vi "Consumer.vi"(8 "error in (no error)":errorcluster, 9 "Data":variant, 10 "Case ID":string, 11 "Scheduler in":refnum<class "Scheduler.lvclass">) -> (0 "error out":errorcluster, 3 "Scheduler out":refnum<class "Scheduler.lvclass">)   [LabVIEW 2020, in "Scheduler.lvlib" / "Scheduler.lvclass"]
uses:
  Scheduler.lvclass
  C:/LabVIEW Code/CIRCUS/TALOS/TALOS_PPL.lvlibp/Father of all uServices/Father of all uServices/Father of all uServices.lvclass
  Scheduler Consumer Case Selector.ctl
  Add RUN Output Data Packet.ctl
  Run Utilities/Schedule Block/Schedule Block.lvclass
  Scheduler.lvclass/Scheduler.ctl
  Run Utilities/Sequence of SBlocks/Sequence of SBlocks.lvclass
  Run Utilities/TypeDefs/Synchronize FPGA Cluster.ctl
  Append Options.ctl
  Run Utilities/TypeDefs/Messages/Schedules With Sync Mask Message.ctl
  Run Utilities/Schedule/Schedule.lvclass
  Run Utilities/TypeDefs/Messages/Append Schedule Message.ctl
  Selection.ctl
  cc9169f9-c1ee-4f38-a286-790ff9248fc5.vi
  7fb8f17a-4757-400c-9638-1f609eaaf37f.vi
  TALOS/TALOS_PPL.lvlibp/Support VIs/Global Memory.vi
  Add RUN Window.vi
  TALOS/TALOS_PPL.lvlibp/Father of all uServices/Father of all uServices/Children Methods/Get GUI Item Value - Variant.vi
  TALOS/TALOS_PPL.lvlibp/Support VIs/Global Constants.vi
  <vilib>/Comparison/Equal/Equal Functor/Equal Functor.lvclass
  TALOS/TALOS_PPL.lvlibp/Father of all uServices/Father of all uServices/Father of all uServices.lvclass
  Run Utilities/Run Utilities.lvlib
  TALOS/TALOS_PPL.lvlibp
  C:/LabVIEW Code/CIRCUS/TALOS/TALOS_PPL.lvlibp/Ancestor/Ancestor/Ancestor.lvclass
  C:/LabVIEW Code/CIRCUS/TALOS/Actor Framework.lvlibp/1abvi3w/vi.lib/ActorFramework/Actor/Actor.lvclass
  C:/LabVIEW Code/CIRCUS/CIRCUS uServices et al/Scheduler/Scheduler.lvclass
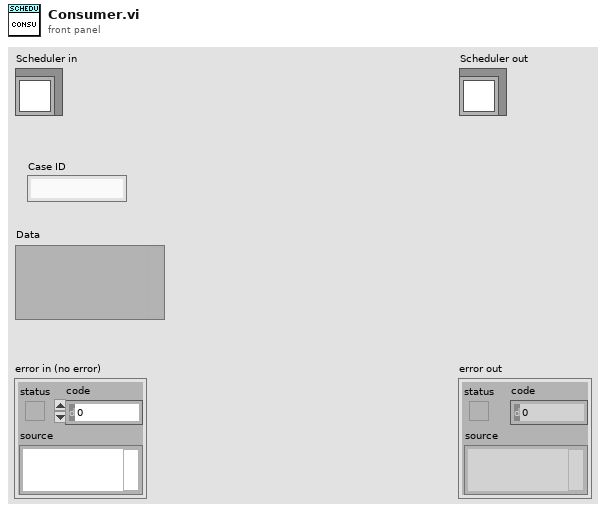
[diagram p1: front panel]
types:
  T1 = typedef "Scheduler.lvlib/Scheduler.lvclass/Scheduler Consumer Case Selector.ctl" = enum16{"Add SBlock", "Update GUI", "Move SBlock", "Select SBlock", "Update Cont.", "Load", "Save", "Reset", "Send to Tamer", "Edit SBlock", "Duplicate SBlock", "Delete SBlock", "Update SBlock", "Init", "Split/Combine Schedules", "Reschedule", "Load Parameters"}
  T2 = enum8{"Enabled", "Disabled", "Disabled and Grayed Out"}
  T3 = typedef "Scheduler.lvlib/Scheduler.lvclass/Add RUN Output Data Packet.ctl" = cluster{"Index":i32, "Schedule Block":refnum<class "Schedule Block.lvclass">}
  T4 = enum32{"Invalid", "Standard", "Closed", "Hidden", "Minimized", "Maximized"}
  T5 = typedef "Scheduler.lvlib/Scheduler.lvclass/Append Options.ctl" = enum16{"New session", "Append to bottom", "Append to top"}
  T6 = typedef "Run Utilities.lvlib/Schedules With Sync Mask Message.ctl" = cluster{"Schedules":refnum<class "Schedule.lvclass">[], "Synchronised":T7[]}
  T7 = typedef "Run Utilities.lvlib/Synchronize FPGA Cluster.ctl" = cluster{"Status":bool, "FPGA Name":string}
  T8 = typedef "Run Utilities.lvlib/Append Schedule Message.ctl" = cluster{"List of FPGAs":set{string}, "Schedules":refnum<class "Schedule.lvclass">[], "To Top?":bool}
  T9 = typedef "Scheduler.lvlib/Scheduler.lvclass/Selection.ctl" = cluster{"Row":i32, "Column":i32}
  T10 = typedef "Run Utilities.lvlib/Sequence of SBlocks.lvclass/Sequence of SBlcoks - GUI.ctl" = cluster{"Total number of scripts":i32, "Time":string, "Sequence of SBlocks":T11[], "Continuous":bool}
  T11 = typedef "Run Utilities.lvlib/Schedule Block.lvclass/Schedule Block - simplified GUI.ctl" = cluster{"Bcg Color":u32, "Index":i32, "No. of runs":i32, "Script name":string, "FPGA name":string, "Parameters":string, "Repetitions":i32}
  T12 = cluster{"SBlock Index":i32, "Sequence Index":i32}
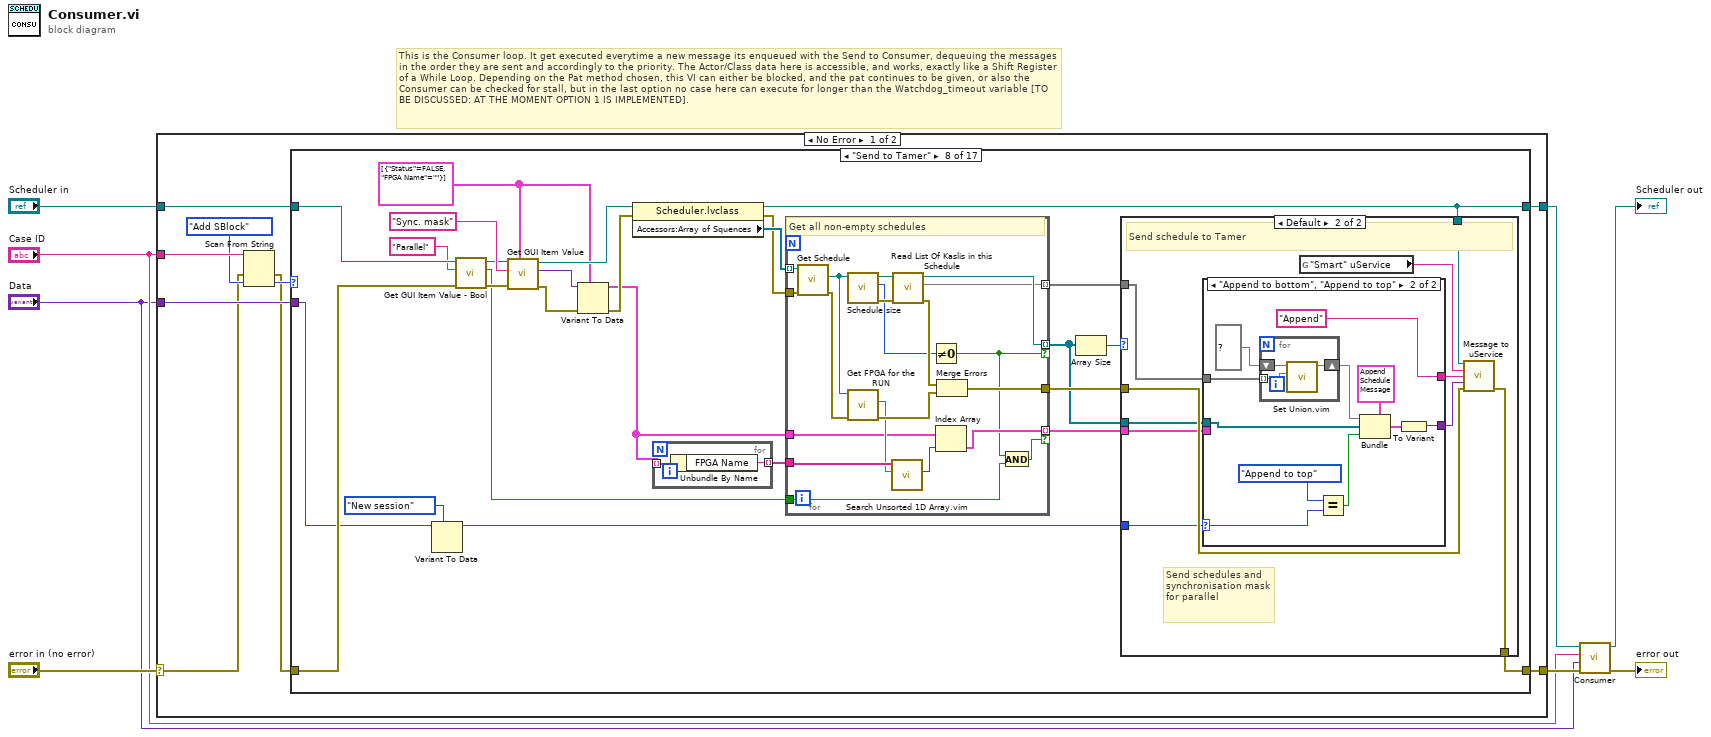
[diagram p0: block diagram]
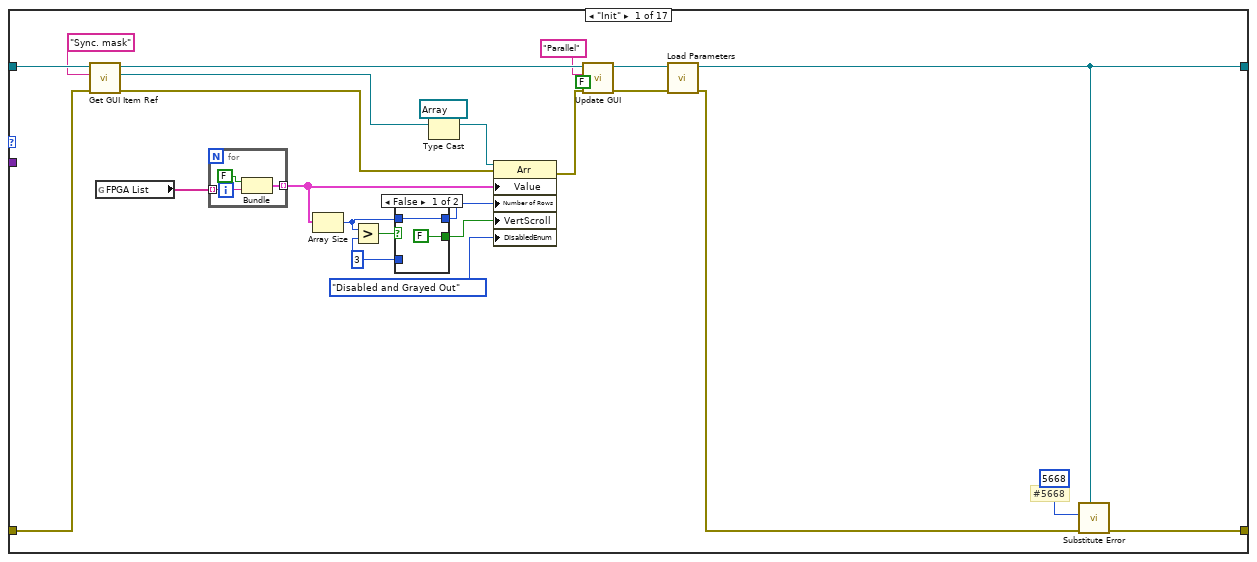
[diagram p2: hidden frame]
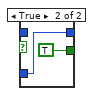
[diagram p3: hidden frame]
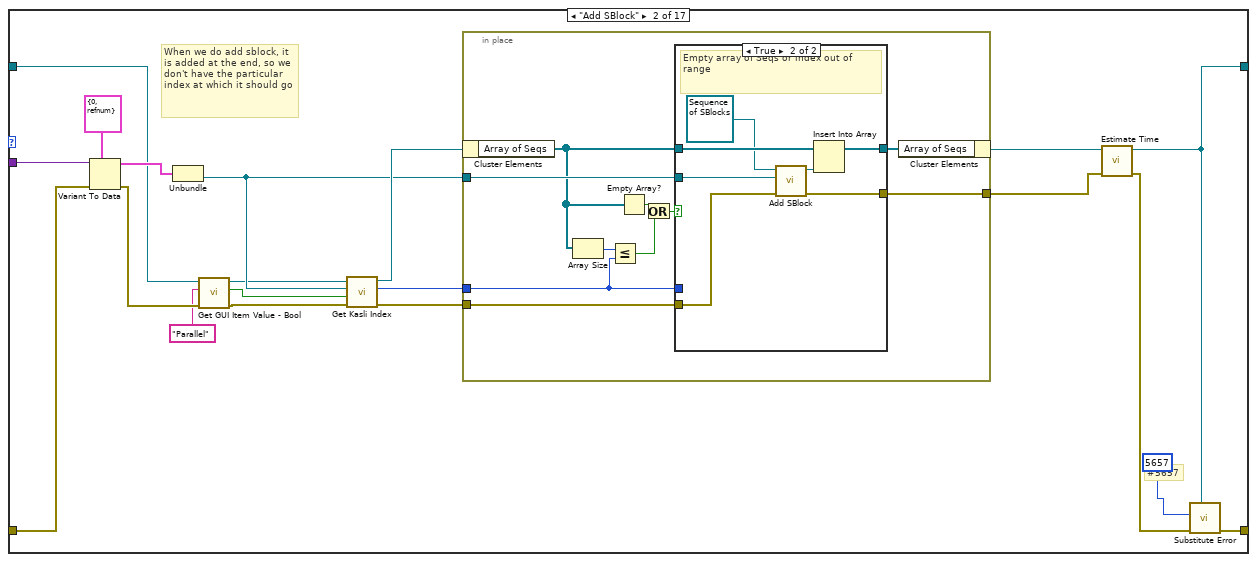
[diagram p4: hidden frame]
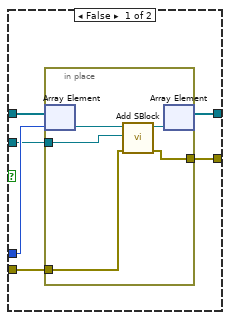
[diagram p5: hidden frame]
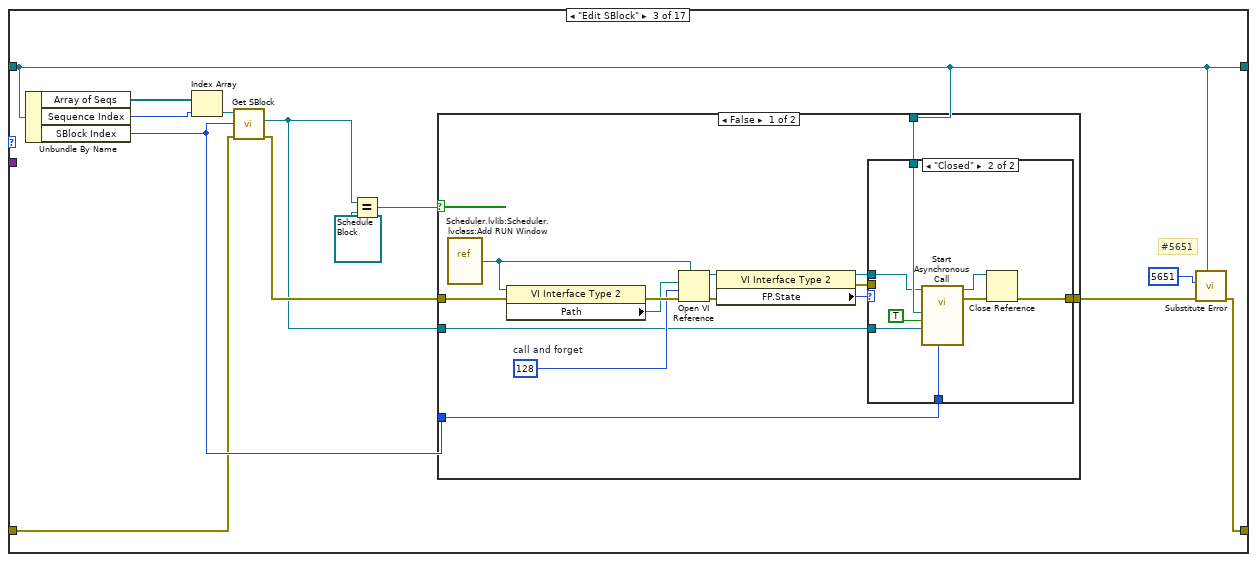
[diagram p6: hidden frame]
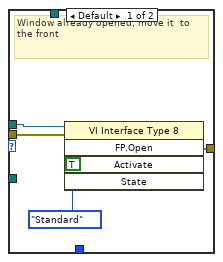
[diagram p7: hidden frame]
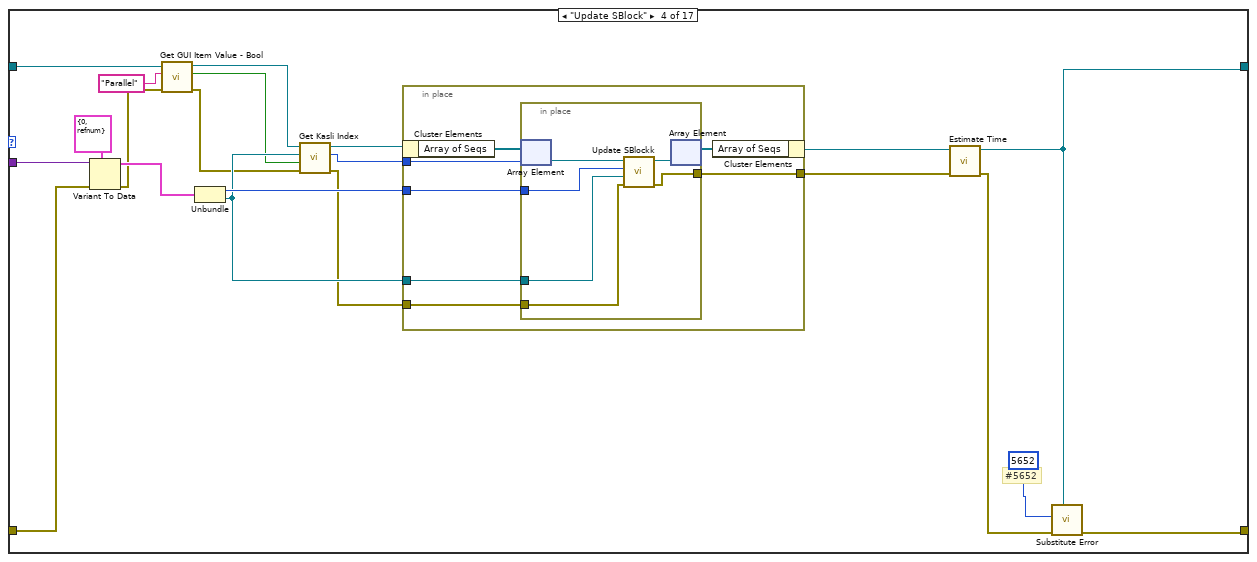
[diagram p9: hidden frame]
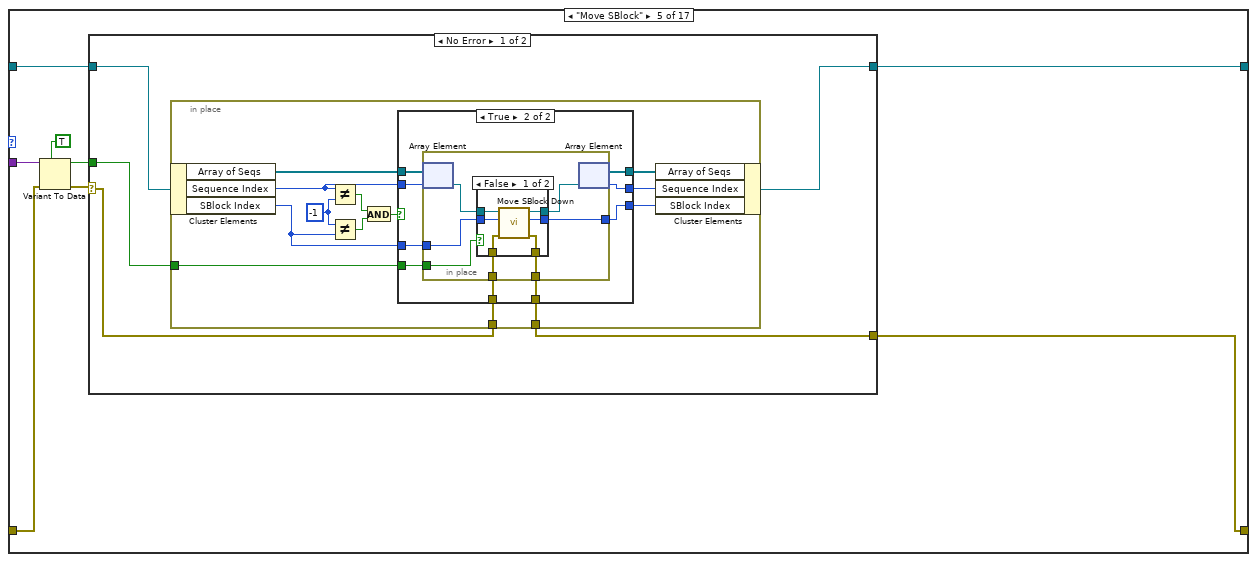
[diagram p10: hidden frame]
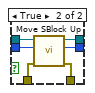
[diagram p12: hidden frame]
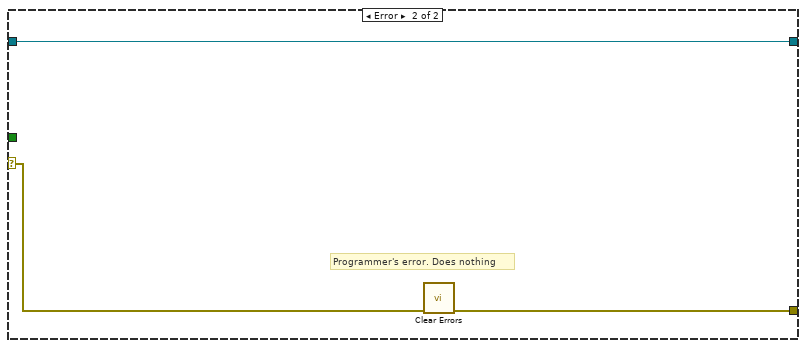
[diagram p13: hidden frame]
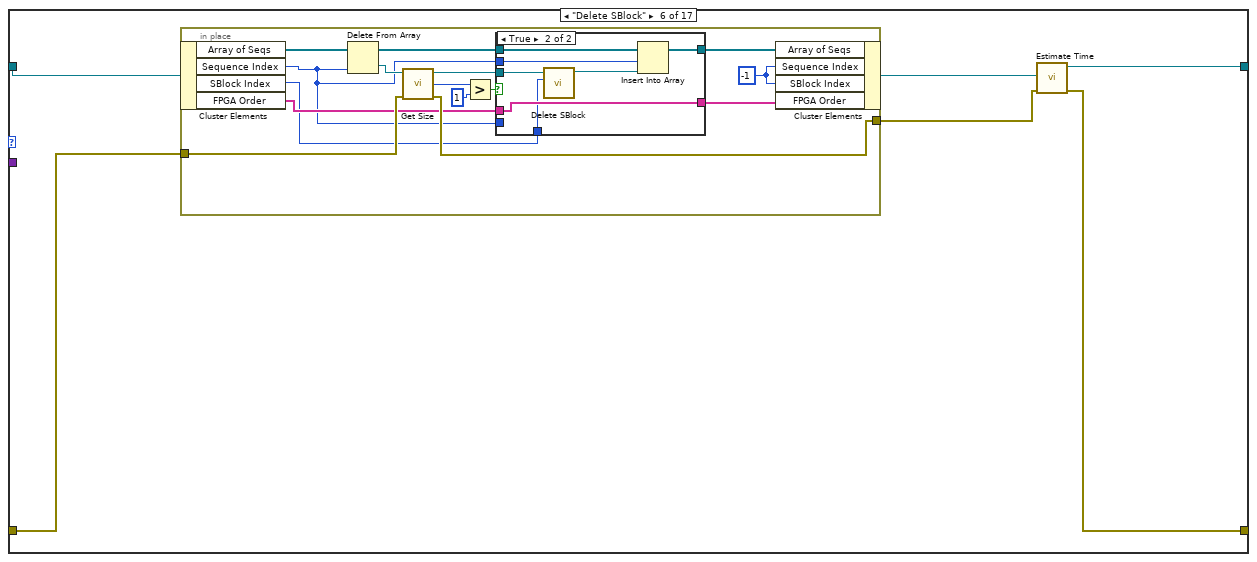
[diagram p14: hidden frame]
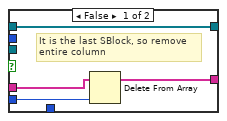
[diagram p15: hidden frame]
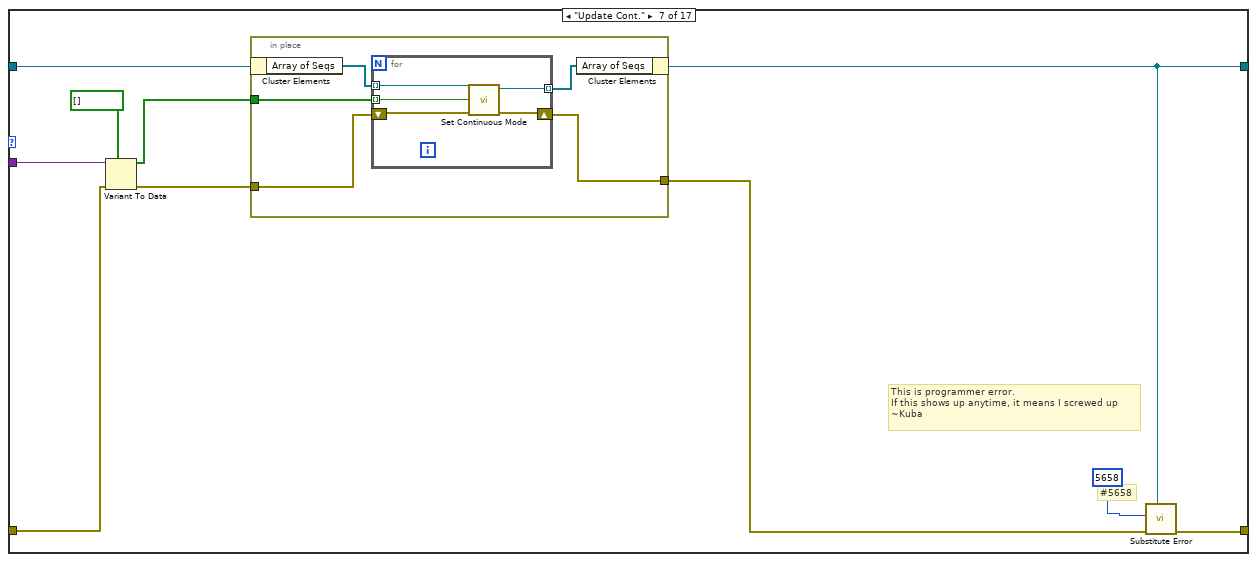
[diagram p16: hidden frame]
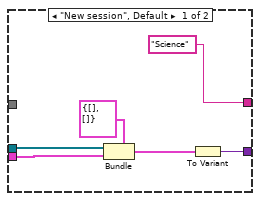
[diagram p18: hidden frame]
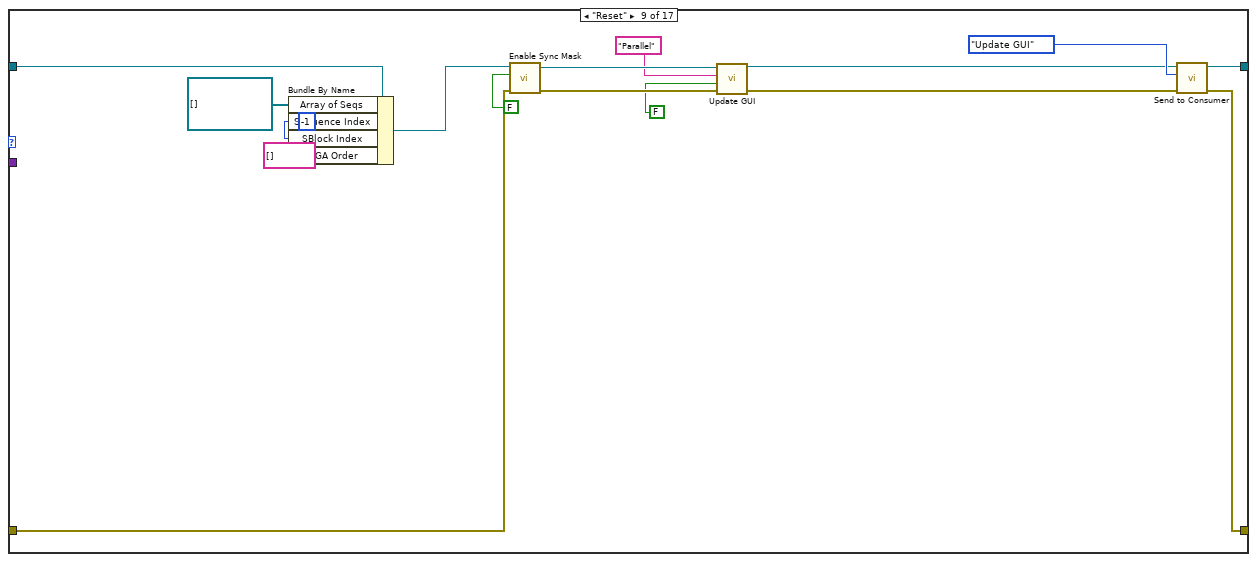
[diagram p19: hidden frame]
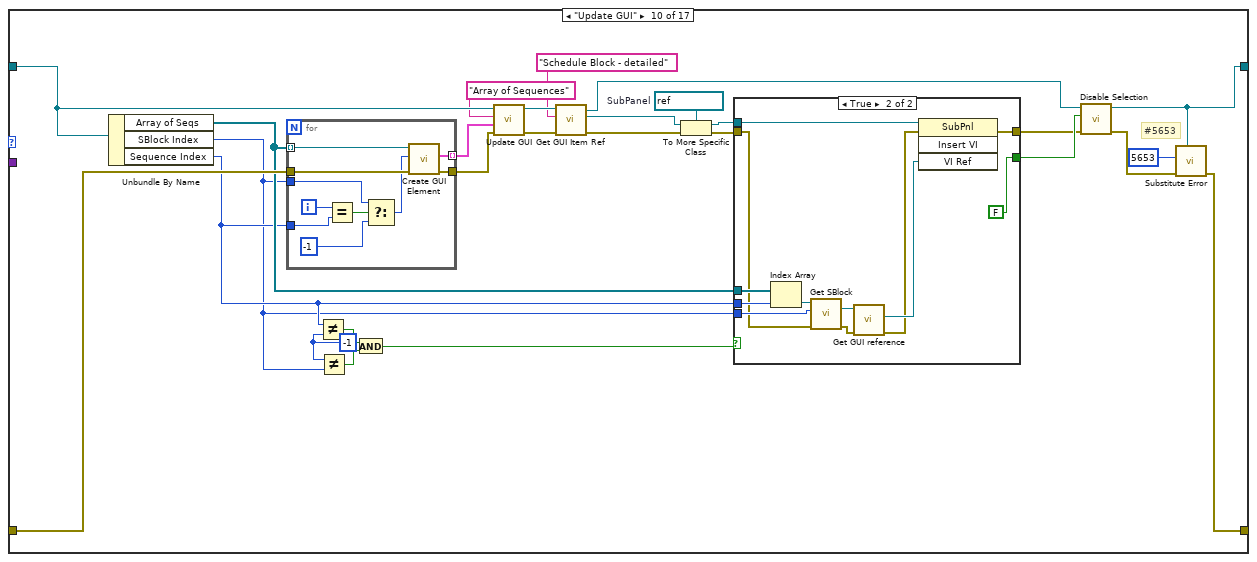
[diagram p20: hidden frame]
diagram:
  # "This is the Consumer loop. It get executed everytime a new message its enqueued with the Send to Consumer, dequeuing the messages in the order they are sent and accordingly to the priority. The Actor/Class data here is accessible, and works, exactly like a Shift Register of a While Loop. Depending on the Pat method chosen, this VI can either be blocked, and the pat continues to be given, or also the Consumer can be checked for stall, but in the last option no case here can execute for longer than the Watchdog_timeout variable [TO BE DISCUSSED: AT THE MOMENT OPTION 1 IS IMPLEMENTED]."
  n1 = case shown="No Error" "error in (no error)" {
    selector: "error in (no error)" -> [w11 w623]
    tunnel: [w10 w624] -> w3
    tunnel: "Scheduler in" -> [w17 w624]
    tunnel: [w15 w623] -> w6
    tunnel: "Case ID" -> [w14 _]
    tunnel: "Data" -> [w16 _]
    frame No Error {
      n2 = Scan From String(input string=w14, error in=w11, default 1=Scheduler_Consumer_Case_Selector."Add SBlock" ("Consumer Case Selector")) -> (error out=w9:errorcluster, output 1=w12:T1)  [unwired: 2 in, 2 out]
      n3 = case shown="\"Send to Tamer\"" w12 {
        tunnel: w17 -> [w35 w55 w108 w143 w180 w239 w275 w305 w371 w405 w437 w489 w517 w540 w586 w616 w621]
        tunnel: w16 -> [_ w69 _ w159 w178 _ w274 w290 _ _ w435 w488 _ w539 w588 w618 _]
        tunnel: [w20 w61 w110 w150 w173 w235 w270 w310 w379 w407 w439 w491 w511 w532 w585 w609 w619] -> w15
        tunnel: w9 -> [w34 w66 w103 w155 w174 w238 w273 w304 w368 w404 w434 w487 w518 w537 w587 w613 w622]
        tunnel: [w19 w58 w108 w147 w179 w236 w269 w309 w380 w394 w438 w490 w512 w536 w583 w610 w620] -> w10
        frame "Init" {
          w37 = 3 ("y")
          # "#5668"
          n4 = call "Get GUI Item Ref.vi"("error in (no error)"=w34, "FP Item Name"="Sync. mask", "uService Template in"=w35) -> ("error out"=w29:errorcluster, "Ctl Refnum"=w33:refnum<vi>, "uService Template out"=w28:refnum<class "Scheduler.lvclass">)  [unwired: 6 in]
          n5 = global read "Global Memory.vi" "FPGA List"() -> (w22:string[])
          n6 = for {
            tunnel: w22 -> [w48] mode=indexing
            tunnel: [w47] -> w36 mode=indexing
            n7 = Bundle(FALSE, "AEgIS PCs List"=w48) -> (w47:cluster{bool, "AEgIS PCs List":string})  [unwired: 1 in]
          }
          n8 = Array Size(array=w36) -> (size(s)=w39:i32)
          n9 = Greater?(x=w39, y=w37) -> (0:w42:bool)
          n10 = case shown="False" w42 {
            tunnel: [w43 w45] -> w41
            tunnel: [FALSE TRUE] -> w40
            tunnel: w39 -> [w43 _]
            tunnel: w37 -> [_ w45]
            frame False {
            }
            frame True {
            }
          }
          n11 = Type Cast(type=refnum<vi> refnum ("reference"), x=w33) -> (*(type *) &x=w31:refnum<vi>)
          n12 = property class="Arr"(reference=w31, error in=w29, "Value"=w36, "Number of Rows"=w41, "VertScroll"=w40, "DisabledEnum"=T2."Disabled and Grayed Out" ("Disabled")) -> (error out=w27:errorcluster)  [unwired: 1 out]
          n13 = call "Update GUI.vi"("error in (no error)"=w27, "Data"=FALSE, "GUI Item Name"="Parallel", "uService Template in"=w28) -> ("error out"=w24:errorcluster, "uService Template out"=w23:refnum<class "Scheduler.lvclass">)  [unwired: 6 in]
          n14 = call-dynamic "Load Parameters.vi"("error in (no error)"=w24, "Scheduler in"=w23) -> ("error out"=w21:errorcluster, "Scheduler out"=w19:refnum<class "Scheduler.lvclass">)  [unwired: 8 in]
          n15 = call "Substitute Error.vi"("LabVIEW Object"=w19, "error in (no error)"=w21, "Error Code"=5668) -> ("error out"=w20:errorcluster)  [unwired: 8 in]
        }
        frame "Add SBlock" {
          # "When we do add sblock, it is added at the end, so we don't have the particular index at which it should go"
          # "#5657"
          n16 = Variant To Data(error in=w66, type=T3 {"Index"=0, "Schedule Block"=refnum} ("Cluster"), Variant=w69) -> (data=w67:T3, error out=w54:errorcluster)
          n17 = Unbundle(w67) -> ("Schedule Block"=w62:refnum<class "Schedule Block.lvclass">)  [unwired: 1 out]
          n18 = call "Get GUI Item Value - Bool.vi"("error in (no error)"=w54, "FP Item Name"="Parallel", "uService Template in"=w55) -> ("error out"=w53:errorcluster, "Value"=w51:bool, "uService Template out"=w52:refnum<class "Scheduler.lvclass">)  [unwired: 6 in]
          n19 = call-dynamic "Get Kasli Index.vi"("error in (no error)"=w53, "Parallel?"=w51, "Schedule Block"=w62, "Scheduler in"=w52) -> ("error out"=w63:errorcluster, "Index"=w64:i32, "Scheduler out"=w65:refnum<class "Scheduler.lvclass">)  [unwired: 5 in]
          n20 = in-place {
            in-place-border: w64 -> [w73]
            in-place-border: w62 -> [w79]
            in-place-border: w63 -> [w77]
            in-place-border: [w76] -> w56
            n21 = in-place-cluster #1(w65) -> ("Array of Seqs"=w71:refnum<class "Sequence of SBlocks.lvclass">[])
            n22 = Array Size(array=w71) -> (size(s)=w74:i32)
            n23 = Less Or Equal?(x=w74, y=w73) -> (x <= y?=w72:bool)
            n24 = Empty Array?(array=w71) -> (empty?=w75:bool)
            n25 = Or(x=w75, y=w72) -> (x .or. y?=w70:bool)
            n26 = case shown="True" w70 {
              tunnel: w73 -> [w85 _]
              tunnel: w71 -> [w84 w97]
              tunnel: w79 -> [w83 w91]
              tunnel: [w82 w96] -> w78
              tunnel: w77 -> [w81 w93]
              tunnel: [w80 w92] -> w76
              frame False {
                n27 = in-place {
                  in-place-border: w83 -> [w87]
                  in-place-border: w81 -> [w88]
                  in-place-border: [w86] -> w80
                  n28 = in-place-array #2(w84, w85) -> (w90:refnum<class "Sequence of SBlocks.lvclass">)
                  n29 = call-dynamic "Add SBlock.vi"("error in (no error)"=w88, "new SBlock"=w87, "Sequence of SBlocks in"=w90) -> ("error out"=w86:errorcluster, "Sequence of SBlocks out"=w89:refnum<class "Sequence of SBlocks.lvclass">)  [unwired: 7 in]
                  n30 = in-place-array #2(w89) -> (w82:refnum<class "Sequence of SBlocks.lvclass">[])  [unwired: 1 out]
                }
              }
              frame True {
                # "Empty array of Seqs or index out of range"
                n31 = call-dynamic "Add SBlock.vi"("error in (no error)"=w93, "new SBlock"=w91, "Sequence of SBlocks in"=refnum<class "Sequence of SBlocks.lvclass"> refnum ("new element/subarray")) -> ("error out"=w92:errorcluster, "Sequence of SBlocks out"=w94:refnum<class "Sequence of SBlocks.lvclass">)  [unwired: 7 in]
                n32 = Insert Into Array(array=w97, new element=w94) -> (w96:refnum<class "Sequence of SBlocks.lvclass">[])  [unwired: 1 in]
              }
            }
            n33 = in-place-cluster #1("Array of Seqs"=w78) -> (w59:refnum<class "Scheduler.lvclass">)
          }
          n34 = call-dynamic "Estimate Time.vi"("error in (no error)"=w56, "Scheduler in"=w59) -> ("error out"=w57:errorcluster, "Scheduler out"=w58:refnum<class "Scheduler.lvclass">)  [unwired: 8 in]
          n35 = call "Substitute Error.vi"("LabVIEW Object"=w58, "error in (no error)"=w57, "Error Code"=5657) -> ("error out"=w61:errorcluster)  [unwired: 8 in]
        }
        frame "Edit SBlock" {
          # "#5651"
          n36 = Unbundle By Name(w108) -> ("Array of Seqs"=w106:refnum<class "Sequence of SBlocks.lvclass">[], "Sequence Index"=w105:i32, "SBlock Index"=w104:i32)
          n37 = Index Array(array=w106, index=w105) -> (element=w102:refnum<class "Sequence of SBlocks.lvclass">)
          n38 = call-dynamic "Get SBlock.vi"("error in (no error)"=w103, "index"=w104, "Sequence of SBlocks in"=w102) -> ("error out"=w101:errorcluster, "Schedule Block"=w98:refnum<class "Schedule Block.lvclass">)  [unwired: 6 in, 1 out]
          n39 = Equal?(x=w98, y=refnum<class "Schedule Block.lvclass"> refnum) -> (x = y?=w99:bool)
          n40 = case shown="False" w99 {
            tunnel: w108 -> [w123 _]
            tunnel: [w122 w138] -> w107
            tunnel: w101 -> [w121 w138]
            tunnel: w104 -> [w120 _]
            tunnel: w98 -> [w115 _]
            frame False {
              w118 = 128  # call and forget
              n41 = vi-ref "Scheduler.lvlib:Scheduler.lvclass:Add RUN Window.vi"() -> (w117:refnum<vi>)
              n42 = property class="VI Interface Type 2"(reference=w117, error in=w121) -> (error out=w124:errorcluster, "Path"=w116:path)  [unwired: 1 out]
              n43 = Open VI Reference(type specifier VI Refnum (for type only)=w117, vi path=w116, options=w118, error in (no error)=w124) -> (vi reference=w119:refnum<vi>, error out=w114:errorcluster)  [unwired: 2 in]
              n44 = property class="VI Interface Type 2"(reference=w119, error in=w114) -> (reference out=w112:refnum<vi>, error out=w111:errorcluster, "FP.State"=w113:T4)
              n45 = case shown="\"Closed\"" w113 {
                tunnel: w123 -> [_ w137]
                tunnel: [w126 w136] -> w122
                tunnel: w120 -> [_ w135]
                tunnel: w115 -> [_ w131]
                tunnel: w112 -> [w125 w130]
                tunnel: w111 -> [w127 _]
                frame Default {
                  # "Window already opened, move it  to the front"
                  n46 = invoke class="VI Interface Type 8" method="FP.Open"(reference=w125, error in=w127, "Activate"=TRUE ("Activate?"), "State"=T4."Standard") -> (error out=w126:errorcluster)  [unwired: 1 in, 4 out]
                }
                frame "Closed" {
                  n47 = call-by-ref "Start Asynchronous Call"(reference=w130, "Index"=w135, "Schedule Block"=w131, "Modify"=TRUE, "CIRCUS_uServices.lvlib:Scheduler.lvlib:Scheduler.lvclass"=w137) -> (reference out=w133:refnum<vi>, error out=w134:errorcluster)  [unwired: 7 in, 2 out]
                  n48 = Close Reference(reference=w133, error in (no error)=w134) -> (error out=w136:errorcluster)
                }
              }
            }
            frame True {
              # "This should never happen, but who am I to know"
              # "Empty SBlock, do nothing"
            }
          }
          n49 = call "Substitute Error.vi"("LabVIEW Object"=w108, "error in (no error)"=w107, "Error Code"=5651) -> ("error out"=w110:errorcluster)  [unwired: 8 in]
        }
        frame "Update SBlock" {
          # "#5652"
          n50 = Variant To Data(error in=w155, type=T3 {"Index"=0, "Schedule Block"=refnum} ("Cluster"), Variant=w159) -> (data=w157:T3, error out=w141:errorcluster)
          n51 = call "Get GUI Item Value - Bool.vi"("error in (no error)"=w141, "FP Item Name"="Parallel", "uService Template in"=w143) -> ("error out"=w140:errorcluster, "Value"=w139:bool, "uService Template out"=w142:refnum<class "Scheduler.lvclass">)  [unwired: 6 in]
          n52 = Unbundle(w157) -> ("Index"=w156:i32, "Schedule Block"=w152:refnum<class "Schedule Block.lvclass">)
          n53 = call-dynamic "Get Kasli Index.vi"("error in (no error)"=w140, "Parallel?"=w139, "Schedule Block"=w152, "Scheduler in"=w142) -> ("error out"=w151:errorcluster, "Index"=w153:i32, "Scheduler out"=w154:refnum<class "Scheduler.lvclass">)  [unwired: 5 in]
          n54 = in-place {
            in-place-border: w156 -> [w162]
            in-place-border: w152 -> [w165]
            in-place-border: w151 -> [w163]
            in-place-border: w153 -> [w161]
            in-place-border: [w160] -> w146
            n55 = in-place-cluster #3(w154) -> ("Array of Seqs"=w166:refnum<class "Sequence of SBlocks.lvclass">[])
            n56 = in-place {
              in-place-border: w165 -> [w171]
              in-place-border: w163 -> [w169]
              in-place-border: w162 -> [w170]
              in-place-border: [w167] -> w160
              n57 = in-place-array #4(w166, w161) -> (w172:refnum<class "Sequence of SBlocks.lvclass">)
              n58 = call-dynamic "Update SBlockk.vi"("error in (no error)"=w169, "element"=w171, "Index"=w170, "Sequence of SBlocks in"=w172) -> ("error out"=w167:errorcluster, "Sequence of SBlocks out"=w168:refnum<class "Sequence of SBlocks.lvclass">)  [unwired: 6 in]
              n59 = in-place-array #4(w168) -> (w164:refnum<class "Sequence of SBlocks.lvclass">[])  [unwired: 1 out]
            }
            n60 = in-place-cluster #3("Array of Seqs"=w164) -> (w148:refnum<class "Scheduler.lvclass">)
          }
          n61 = call-dynamic "Estimate Time.vi"("error in (no error)"=w146, "Scheduler in"=w148) -> ("error out"=w145:errorcluster, "Scheduler out"=w147:refnum<class "Scheduler.lvclass">)  [unwired: 8 in]
          n62 = call "Substitute Error.vi"("LabVIEW Object"=w147, "error in (no error)"=w145, "Error Code"=5652) -> ("error out"=w150:errorcluster)  [unwired: 8 in]
        }
        frame "Move SBlock" {
          n63 = Variant To Data(error in=w174, type=TRUE, Variant=w178) -> (data=w176:bool, error out=w175:errorcluster)
          n64 = case shown="No Error" w175 {
            selector: w175 -> [w182 w232]
            tunnel: w180 -> [w185 w233]
            tunnel: [w184 w233] -> w179
            tunnel: w176 -> [w183 _]
            tunnel: [w181 w231] -> w173
            frame No Error {
              n65 = in-place {
                in-place-border: w182 -> [w194]
                in-place-border: [w193] -> w181
                in-place-border: w183 -> [w186]
                w198 = -1 ("y")
                n66 = in-place-cluster #5(w185) -> ("Array of Seqs"=w192:refnum<class "Sequence of SBlocks.lvclass">[], "Sequence Index"=w191:i32, "SBlock Index"=w190:i32)
                n67 = Not Equal?(x=w191, y=w198) -> (x != y?=w196:bool)
                n68 = Not Equal?(x=w198, y=w190) -> (x != y?=w197:bool)
                n69 = And(x=w196, y=w197) -> (x .and. y?=w195:bool)
                n70 = case shown="True" w195 {
                  tunnel: w192 -> [w199 w211]
                  tunnel: w191 -> [w200 w210]
                  tunnel: w190 -> [w201 w209]
                  tunnel: w194 -> [w202 w208]
                  tunnel: [w202 w207] -> w193
                  tunnel: [w199 w206] -> w189
                  tunnel: [w200 w205] -> w188
                  tunnel: [w201 w204] -> w187
                  tunnel: w186 -> [_ w203]
                  frame False {
                  }
                  frame True {
                    n71 = in-place {
                      in-place-border: w209 -> [w217]
                      in-place-border: w208 -> [w216]
                      in-place-border: [w214] -> w204
                      in-place-border: [w213] -> w207
                      in-place-border: w203 -> [w212]
                      n72 = in-place-array #6(w211, w210) -> (w218:refnum<class "Sequence of SBlocks.lvclass">)
                      n73 = case shown="False" w212 {
                        tunnel: w218 -> [w224 w230]
                        tunnel: w217 -> [w223 w229]
                        tunnel: w216 -> [w222 w228]
                        tunnel: [w219 w227] -> w215
                        tunnel: [w220 w226] -> w214
                        tunnel: [w221 w225] -> w213
                        frame False {
                          n74 = call-dynamic "Move SBlock Down.vi"("error in (no error)"=w222, "index"=w223, "Sequence of SBlocks in"=w224) -> ("error out"=w221:errorcluster, "New Index"=w220:i32, "Sequence of SBlocks out"=w219:refnum<class "Sequence of SBlocks.lvclass">)  [unwired: 6 in]
                        }
                        frame True {
                          n75 = call-dynamic "Move SBlock Up.vi"("error in (no error)"=w228, "index"=w229, "Sequence of SBlocks in"=w230) -> ("error out"=w225:errorcluster, "New Index"=w226:i32, "Sequence of SBlocks out"=w227:refnum<class "Sequence of SBlocks.lvclass">)  [unwired: 6 in]
                        }
                      }
                      n76 = in-place-array #6(w215) -> (w206:refnum<class "Sequence of SBlocks.lvclass">[], w205:i32)
                    }
                  }
                }
                n77 = in-place-cluster #5("Array of Seqs"=w189, "Sequence Index"=w188, "SBlock Index"=w187) -> (w184:refnum<class "Scheduler.lvclass">)
              }
            }
            frame Error {
              # "Programmer's error. Does nothing"
              n78 = call <vilib>:"Clear Errors.vi"("error in (no error)"=w232) -> ("error out"=w231:errorcluster)  [unwired: 5 in, 1 out]
            }
          }
        }
        frame "Delete SBlock" {
          n79 = in-place {
            in-place-border: w238 -> [w251]
            in-place-border: [w246] -> w234
            w254 = -1 ("Sequence Index")
            n80 = in-place-cluster #7(w239) -> ("Array of Seqs"=w253:refnum<class "Sequence of SBlocks.lvclass">[], "Sequence Index"=w242:i32, "SBlock Index"=w241:i32, "FPGA Order"=w244:string[])
            n81 = Delete From Array(array=w253, index=w242) -> (deleted portion=w245:refnum<class "Sequence of SBlocks.lvclass">, array with subset deleted=w240:refnum<class "Sequence of SBlocks.lvclass">[])  [unwired: 1 in]
            n82 = call-dynamic "Get Size.vi"("error in (no error)"=w251, "Sequence of SBlocks in"=w245) -> ("error out"=w246:errorcluster, "size"=w250:i32, "Sequence of SBlocks out"=w252:refnum<class "Sequence of SBlocks.lvclass">)  [unwired: 7 in]
            n83 = Greater?(x=w250, y=1) -> (0:w247:bool)
            n84 = case shown="True" w247 {
              tunnel: w240 -> [w258 w265]
              tunnel: w252 -> [_ w261]
              tunnel: w242 -> [_ w264]
              tunnel: [w258 w263] -> w248
              tunnel: w244 -> [w257 w262]
              tunnel: w242 -> [w256 _]
              tunnel: [w255 w262] -> w243
              tunnel: w241 -> [_ w260]
              frame False {
                # "It is the last SBlock, so remove entire column"
                n85 = Delete From Array(array=w257, index=w256) -> (array with subset deleted=w255:string[])  [unwired: 1 in, 1 out]
              }
              frame True {
                n86 = call-dynamic "Delete SBlock.vi"("index"=w260, "Sequence of SBlocks in"=w261) -> ("Sequence of SBlocks out"=w259:refnum<class "Sequence of SBlocks.lvclass">)  [unwired: 7 in, 2 out]
                n87 = Insert Into Array(array=w265, index=w264, new element=w259) -> (w263:refnum<class "Sequence of SBlocks.lvclass">[])
              }
            }
            n88 = in-place-cluster #7("Array of Seqs"=w248, "Sequence Index"=w254, "SBlock Index"=w254, "FPGA Order"=w243) -> (w237:refnum<class "Scheduler.lvclass">)
          }
          n89 = call-dynamic "Estimate Time.vi"("error in (no error)"=w234, "Scheduler in"=w237) -> ("error out"=w235:errorcluster, "Scheduler out"=w236:refnum<class "Scheduler.lvclass">)  [unwired: 8 in]
        }
        frame "Update Cont." {
          # "This is programmer error.\nIf this shows up anytime, it means I screwed up\n~Kuba"
          # "#5658"
          n90 = Variant To Data(error in=w273, type=bool[] [], Variant=w274) -> (data=w266:bool[], error out=w272:errorcluster)
          n91 = in-place {
            in-place-border: w272 -> [w280]
            in-place-border: [w279] -> w271
            in-place-border: w266 -> [w277]
            n92 = in-place-cluster #8(w275) -> ("Array of Seqs"=w278:refnum<class "Sequence of SBlocks.lvclass">[])
            n93 = for {
              shift-right: [w284] -> w279
              shift-left: w280 -> [w285]
              tunnel: w278 -> [w283] mode=indexing
              tunnel: w277 -> [w282] mode=indexing
              tunnel: [w281] -> w276 mode=indexing
              n94 = call-dynamic "Set Continuous Mode.vi"("error in (no error)"=w285, "Continuous?"=w282, "Sequence of SBlocks in"=w283) -> ("error out"=w284:errorcluster, "Sequence of SBlocks out"=w281:refnum<class "Sequence of SBlocks.lvclass">)  [unwired: 7 in]
            }
            n95 = in-place-cluster #8("Array of Seqs"=w276) -> (w269:refnum<class "Scheduler.lvclass">)
          }
          n96 = call "Substitute Error.vi"("LabVIEW Object"=w269, "error in (no error)"=w271, "Error Code"=5658) -> ("error out"=w270:errorcluster)  [unwired: 8 in]
        }
        frame "Send to Tamer" {
          w292 = T7[] [{"Status"=FALSE, "FPGA Name"=""}]
          n97 = Variant To Data(type=Append_Options."New session" ("Append"), Variant=w290) -> (data=w287:T5)  [unwired: 1 in, 1 out]
          n98 = call "Get GUI Item Value - Bool.vi"("error in (no error)"=w304, "FP Item Name"="Parallel", "uService Template in"=w305) -> ("error out"=w302:errorcluster, "Value"=w291:bool, "uService Template out"=w293:refnum<class "Scheduler.lvclass">)  [unwired: 6 in]
          n99 = call-poly "Get GUI Item Value.vi"("Default"=w292, "error in (no error)"=w302, "FP Item Name"="Sync. mask", "uService Template in"=w293) -> ("error out"=w299:errorcluster, "Value"=w300:variant, "uService Template out"=w298:refnum<class "Scheduler.lvclass">)  [unwired: 5 in]
          n100 = Variant To Data(error in=w299, type=w292, Variant=w300) -> (data=w288:T7[], error out=w297:errorcluster)
          n101 = property class="Scheduler.lvclass"(reference=w298, error in=w297) -> (reference out=w309:refnum<class "Scheduler.lvclass">, error out=w307:errorcluster, "Accessors:Array of Squences"=w308:refnum<class "Sequence of SBlocks.lvclass">[])
          n102 = for {
            tunnel: w288 -> [w313] mode=indexing
            tunnel: [w312] -> w295 mode=indexing
            n103 = Unbundle By Name(w313) -> ("FPGA Name"=w312:string)
          }
          n104 = for {
            tunnel: [w324] -> w311
            tunnel: [w315] -> w296 mode=indexing if=w323
            tunnel: w308 -> [w332] mode=indexing
            tunnel: w307 -> [w331]
            tunnel: w288 -> [w327]
            tunnel: w295 -> [w329]
            tunnel: [w325] -> w294 mode=indexing if=w321
            tunnel: w291 -> [w322]
            tunnel: [w314] -> w286 mode=indexing
            # "Get all non-empty schedules"
            n105 = call-dynamic "Get Schedule.vi"("error in (no error)"=w331, "Sequence of SBlocks in"=w332) -> ("error out"=w333:errorcluster, "Schedule"=w320:refnum<class "Schedule.lvclass">)  [unwired: 7 in, 1 out]
            n106 = call-dynamic "Schedule size.vi"("Schedule in"=w320) -> ("error out"=w318:errorcluster, "Size"=w316:i32, "Schedule out"=w319:refnum<class "Schedule.lvclass">)  [unwired: 8 in]
            n107 = call-dynamic "Get FPGA for the RUN.vi"("error in (no error)"=w333, "Schedule in"=w320) -> ("error out"=w330:errorcluster, "FPGA Name"=w328:string)  [unwired: 7 in, 1 out]
            n108 = call "Search Unsorted 1D Array.vim"("element"=w328, "unsorted 1D array"=w329) -> ("index of element"=w326:i32)  [unwired: 9 in]
            n109 = call-dynamic "Read List Of Kaslis in this Schedule.vi"("error in (no error)"=w318, "Schedule in"=w319) -> ("error out"=w317:errorcluster, "List of FPGAs"=w314:set{string}, "Schedule out"=w315:refnum<class "Schedule.lvclass">)  [unwired: 7 in]
            n110 = Not Equal To 0?(x=w316) -> (x != 0?=w323:bool)
            n111 = Index Array(array=w327, index=w326) -> (element=w325:T7)
            n112 = Merge Errors(w317, w330) -> (w324:errorcluster)
            n113 = And(x=w323, y=w322) -> (x .and. y?=w321:bool)
          }
          n114 = Array Size(array=w296) -> (size(s)=w306:i32)
          n115 = case shown="Default" w306 {
            tunnel: w309 -> [_ w343]
            tunnel: [w334 w342] -> w310
            tunnel: w311 -> [w334 w344]
            tunnel: w296 -> [_ w336]
            tunnel: w294 -> [_ w335]
            tunnel: w287 -> [_ w340]
            tunnel: w286 -> [_ w337]
            frame 0 {
              # "There are no non-empty schedules, do nothing"
            }
            frame Default {
              # "Send schedules and synchronisation mask for parallel"
              # "Send schedule to Tamer"
              n116 = case shown="\"Append to bottom\", \"Append to top\"" w340 {
                selector: w340 -> [_ w356]
                tunnel: ["Science" ("Message") "Append" ("Message")] -> w339
                tunnel: [w349 w358] -> w338
                tunnel: w337 -> [_ w361]
                tunnel: w336 -> [w348 w351]
                tunnel: w335 -> [w347 _]
                frame "New session", Default {
                  n117 = Bundle(cluster=T6 {"Schedules"=[], "Synchronised"=[]}, "Schedules"=w348, "Synchronised"=w347) -> (w345:T6)
                  n118 = To Variant(anything=w345) -> (Variant=w349:variant)
                }
                frame "Append to bottom", "Append to top" {
                  n119 = for {
                    tunnel: w361 -> [w363] mode=indexing
                    shift-right: [w362] -> w359
                    shift-left: set{string} {} ("List of FPGAs") -> [w364]
                    n120 = call "Set Union.vim"("set 2"=w363, "set 1"=w364) -> ("union"=w362:set{string})  [unwired: 9 in]
                  }
                  n121 = Equal?(x=Append_Options."Append to top", y=w356) -> (x = y?=w354:bool)
                  n122 = Bundle(cluster=T8 {"List of FPGAs"={}, "Schedules"=[], "To Top?"=FALSE} ("Schedule message"), "List of FPGAs"=w359, "Schedules"=w351, "To Top?"=w354) -> (w357:T8)
                  n123 = To Variant(anything=w357) -> (Variant=w358:variant)
                }
              }
              n124 = global read "Global Constants.vi" "\"Smart\" uService"() -> (w341:string)
              n125 = call "Message to uService.vi"("Father of all uServices in"=w343, "uService ID"=w341, "Message"=w339, "Data"=w338, "error in (no error)"=w344) -> ("error out"=w342:errorcluster)  [unwired: 9 in, 1 out]
            }
          }
        }
        frame "Reset" {
          w367 = -1 ("Sequence Index")
          n126 = Bundle By Name(cluster=w371, "Array of Seqs"=refnum<class "Sequence of SBlocks.lvclass">[] [] ("Array of Squences"), "Sequence Index"=w367, "SBlock Index"=w367, "FPGA Order"=string[] [] ("Kasli Order")) -> (w369:refnum<class "Scheduler.lvclass">)
          n127 = call-dynamic "Enable Sync Mask.vi"("error in (no error)"=w368, "Enable"=FALSE, "Scheduler in"=w369) -> ("error out"=w377:errorcluster, "Scheduler out"=w376:refnum<class "Scheduler.lvclass">)  [unwired: 7 in]
          n128 = call "Update GUI.vi"("error in (no error)"=w377, "Data"=FALSE, "GUI Item Name"="Parallel", "uService Template in"=w376) -> ("error out"=w375:errorcluster, "uService Template out"=w365:refnum<class "Scheduler.lvclass">)  [unwired: 6 in]
          n129 = call "Send to Consumer.vi"("error in (no error)"=w375, "Case ID"=Scheduler_Consumer_Case_Selector."Update GUI" ("Consumer Case Selector"), "uService Template in"=w365) -> ("error out"=w379:errorcluster, "uService Template out"=w380:refnum<class "Scheduler.lvclass">)  [unwired: 7 in]
        }
        frame "Update GUI" {
          w383 = refnum<vi> refnum  # SubPanel
          w395 = -1 ("y")
          # "#5653"
          n130 = Unbundle By Name(w405) -> ("Array of Seqs"=w401:refnum<class "Sequence of SBlocks.lvclass">[], "SBlock Index"=w396:i32, "Sequence Index"=w397:i32)
          n131 = for {
            tunnel: w401 -> [w433] mode=indexing
            tunnel: w404 -> [w432]
            tunnel: w397 -> [w430]
            tunnel: w396 -> [w428]
            tunnel: [w425] -> w403 mode=indexing
            tunnel: [w424] -> w402
            i -> [w429]
            n132 = Equal?(x=w429, y=w430) -> (x = y?=w431:bool)
            n133 = Select(t=w428, s=w431, f=-1) -> (s? t:f=w426:i32)
            n134 = call-dynamic "Create GUI Element.vi"("error in (no error)"=w432, "Highlight index"=w426, "Sequence of SBlocks in"=w433) -> ("error out"=w424:errorcluster, "Sequence of SBlocks - GUI"=w425:T10)  [unwired: 6 in, 1 out]
          }
          n135 = Not Equal?(x=w397, y=w395) -> (x != y?=w400:bool)
          n136 = Not Equal?(x=w395, y=w396) -> (x != y?=w399:bool)
          n137 = And(x=w400, y=w399) -> (x .and. y?=w398:bool)
          n138 = call "Update GUI.vi"("error in (no error)"=w402, "Data"=w403, "GUI Item Name"="Array of Sequences", "uService Template in"=w405) -> ("error out"=w389:errorcluster, "uService Template out"=w390:refnum<class "Scheduler.lvclass">)  [unwired: 6 in]
          n139 = call "Get GUI Item Ref.vi"("error in (no error)"=w389, "FP Item Name"="Schedule Block - detailed", "uService Template in"=w390) -> ("error out"=w385:errorcluster, "Ctl Refnum"=w384:refnum<vi>, "uService Template out"=w386:refnum<class "Scheduler.lvclass">)  [unwired: 6 in]
          n140 = To More Specific Class(target class=w383, reference=w384, error in=w385) -> (specific class reference=w382:refnum<vi>, error out=w381:errorcluster)
          n141 = case shown="True" w398 {
            tunnel: w401 -> [_ w423]
            tunnel: w397 -> [_ w422]
            tunnel: w396 -> [_ w420]
            tunnel: [w408 w414] -> w391
            tunnel: w381 -> [w409 w416]
            tunnel: [TRUE ("Disable?") FALSE ("Disable?")] -> w392
            tunnel: w382 -> [w410 w415]
            frame False {
              n142 = invoke class="SubPnl" method="Remove VI"(reference=w410, error in=w409) -> (error out=w408:errorcluster)  [unwired: 1 in, 2 out]
            }
            frame True {
              n143 = Index Array(array=w423, index=w422) -> (element=w421:refnum<class "Sequence of SBlocks.lvclass">)
              n144 = call-dynamic "Get SBlock.vi"("error in (no error)"=w416, "index"=w420, "Sequence of SBlocks in"=w421) -> ("error out"=w418:errorcluster, "Schedule Block"=w419:refnum<class "Schedule Block.lvclass">)  [unwired: 6 in, 1 out]
              n145 = call-dynamic "Get GUI reference.vi"("error in (no error)"=w418, "Schedule Block in"=w419) -> ("error out"=w412:errorcluster, "This VI"=w413:refnum<vi>)  [unwired: 7 in, 1 out]
              n146 = invoke class="SubPnl" method="Insert VI"(reference=w415, error in=w412, "VI Ref"=w413) -> (error out=w414:errorcluster)  [unwired: 1 in, 3 out]
            }
          }
          n147 = call-dynamic "Disable Selection.vi"("error in (no error)"=w391, "Disable?"=w392, "Scheduler in"=w386) -> ("error out"=w393:errorcluster, "Scheduler out"=w394:refnum<class "Scheduler.lvclass">)  [unwired: 7 in]
          n148 = call "Substitute Error.vi"("LabVIEW Object"=w394, "error in (no error)"=w393, "Error Code"=5653) -> ("error out"=w407:errorcluster)  [unwired: 8 in]
        }
        frame "Load" {
          n149 = Variant To Data(error in=w434, type=refnum<file> refnum ("refnum out"), Variant=w435) -> (data=w441:refnum<file>, error out=w442:errorcluster)
          n150 = case shown="No Error" w442 {
            selector: w442 -> [w465 w485]
            tunnel: w437 -> [w455 w484]
            tunnel: [w464 w484] -> w438
            tunnel: w441 -> [w466 _]
            tunnel: [w451 w485] -> w440
            frame No Error {
              n151 = Read from Text File(file (use dialog)=w466, error in=w465) -> (refnum out=w461:refnum<file>, text=w458:string, error out=w462:errorcluster)  [unwired: 2 in, 1 out]
              n152 = Unflatten From XML(xml string=w458, type=refnum<class "Sequence of SBlocks.lvclass">[] [] ("Array of Seqs"), error in (no error)=w462) -> (value=w459:refnum<class "Sequence of SBlocks.lvclass">[], error out=w460:errorcluster)
              n153 = case shown="Error .." w460 {
                selector: w460 -> [w469 w477]
                tunnel: [w469 w470] -> w453
                tunnel: w459 -> [w468 _]
                tunnel: [w468 w471] -> w454
                tunnel: w458 -> [_ w476]
                frame No Error {
                }
                frame Error {
                  # "Error, maybe trying to read a file in the old format"
                  n154 = call <vilib>:"Clear Errors.vi"("error in (no error)"=w477) -> ("error out"=w475:errorcluster)  [unwired: 5 in, 1 out]
                  n155 = Unflatten From XML(xml string=w476, type=refnum<class "Schedule.lvclass"> refnum ("CIRCUS_uServices.lvlib:Run Utilities.lvlib:Schedule.lvclass"), error in (no error)=w475) -> (value=w472:refnum<class "Schedule.lvclass">, error out=w473:errorcluster)
                  n156 = case shown="Error .." w473 {
                    selector: w473 -> [_ w483]
                    tunnel: w472 -> [w481 _]
                    tunnel: [w479 refnum<class "Sequence of SBlocks.lvclass">[] []] -> w471
                    tunnel: [w478 w483] -> w470
                    frame No Error {
                      n157 = call "Convert Schedule to Sequence of SBlocks.vi"("Schedule"=w481) -> ("error out"=w478:errorcluster, "Sequence of SBlocks"=w480:refnum<class "Sequence of SBlocks.lvclass">)  [unwired: 1 in]
                      n158 = Build Array(w480) -> (w479:refnum<class "Sequence of SBlocks.lvclass">[])
                    }
                    frame Error {
                    }
                  }
                }
              }
              n159 = Close File(refnum=w461) -> (error out=w467:errorcluster)  [unwired: 1 in, 1 out]
              n160 = call-dynamic "Append Loaded Sequences.vi"("error in (no error)"=w453, "Array of Seqs Loaded"=w454, "Scheduler in"=w455) -> ("error out"=w452:errorcluster, "Scheduler out"=w456:refnum<class "Scheduler.lvclass">)  [unwired: 7 in]
              n161 = call-dynamic "Estimate Time.vi"("error in (no error)"=w452, "Scheduler in"=w456) -> ("error out"=w463:errorcluster, "Scheduler out"=w449:refnum<class "Scheduler.lvclass">)  [unwired: 8 in]
              n162 = call "Send to Consumer.vi"("error in (no error)"=w463, "Case ID"=Scheduler_Consumer_Case_Selector."Update GUI" ("Consumer Case Selector"), "uService Template in"=w449) -> ("error out"=w450:errorcluster, "uService Template out"=w464:refnum<class "Scheduler.lvclass">)  [unwired: 7 in]
              n163 = Merge Errors(w467, w450) -> (w451:errorcluster)
            }
            frame Error {
            }
          }
          n164 = case shown="No Error" w440 {
            selector: w440 -> [w443 w447]
            tunnel: [w443 w446] -> w439
            frame No Error {
            }
            frame Error {
              n165 = call <vilib>:"Clear Errors.vi"("error in (no error)"=w447) -> ("error out"=w444:errorcluster)  [unwired: 5 in, 1 out]
              n166 = call "Temporised Pop-up Window.vi"("error in (no error)"=w444, "Text"="Error while loading sequence from the file!") -> ("error out"=w446:errorcluster)  [unwired: 9 in]
            }
          }
        }
        frame "Save" {
          n167 = Variant To Data(error in=w487, type=refnum<file> refnum ("refnum out"), Variant=w488) -> (data=w493:refnum<file>, error out=w494:errorcluster)
          n168 = case shown="Error .." w494 {
            selector: w494 -> [w500 w510]
            tunnel: w489 -> [w505 w509]
            tunnel: [w505 w509] -> w490
            tunnel: w493 -> [w501 _]
            tunnel: [w507 w510] -> w492
            frame No Error {
              n169 = property class="Scheduler.lvclass"(reference=w505) -> ("Accessors:Array of Squences"=w502:refnum<class "Sequence of SBlocks.lvclass">[])  [unwired: 1 in, 2 out]
              n170 = Flatten To XML(6:w502) -> (2:w503:string)
              n171 = Write to Text File(file (use dialog)=w501, text=w503, error in=w500) -> (refnum out=w504:refnum<file>, error out=w506:errorcluster)  [unwired: 1 in, 1 out]
              n172 = Close File(refnum=w504) -> (error out=w508:errorcluster)  [unwired: 1 in, 1 out]
              n173 = Merge Errors(w508, w506) -> (w507:errorcluster)
            }
            frame Error {
            }
          }
          n174 = case shown="No Error" w492 {
            selector: w492 -> [w495 w499]
            tunnel: [w495 w498] -> w491
            frame No Error {
            }
            frame Error {
              n175 = call <vilib>:"Clear Errors.vi"("error in (no error)"=w499) -> ("error out"=w496:errorcluster)  [unwired: 5 in, 1 out]
              n176 = call "Temporised Pop-up Window.vi"("error in (no error)"=w496, "Text"="Error while saving the sequence in the file!") -> ("error out"=w498:errorcluster)  [unwired: 9 in]
            }
          }
        }
        frame "Duplicate SBlock" {
          n177 = Unbundle By Name(w517) -> ("Sequence Index"=w516:i32, "SBlock Index"=w515:i32)
          n178 = in-place {
            in-place-border: w518 -> [w523]
            in-place-border: w516 -> [w521]
            in-place-border: w515 -> [w520]
            in-place-border: [w519] -> w514
            n179 = in-place-cluster #9(w517) -> ("Array of Seqs"=w524:refnum<class "Sequence of SBlocks.lvclass">[])
            n180 = in-place {
              in-place-border: w520 -> [w528]
              in-place-border: w523 -> [w526]
              in-place-border: [w525] -> w519
              n181 = in-place-array #10(w524, w521) -> (w529:refnum<class "Sequence of SBlocks.lvclass">)
              n182 = call-dynamic "Duplicate SBlock.vi"("error in (no error)"=w526, "index"=w528, "Sequence of SBlocks in"=w529) -> ("error out"=w525:errorcluster, "Sequence of SBlocks out"=w527:refnum<class "Sequence of SBlocks.lvclass">)  [unwired: 7 in]
              n183 = in-place-array #10(w527) -> (w522:refnum<class "Sequence of SBlocks.lvclass">[])  [unwired: 1 out]
            }
            n184 = in-place-cluster #9("Array of Seqs"=w522) -> (w513:refnum<class "Scheduler.lvclass">)
          }
          n185 = call-dynamic "Estimate Time.vi"("error in (no error)"=w514, "Scheduler in"=w513) -> ("error out"=w511:errorcluster, "Scheduler out"=w512:refnum<class "Scheduler.lvclass">)  [unwired: 8 in]
        }
        frame "Select SBlock" {
          # "This is a programmer's error"
          # "#5659"
          n186 = Variant To Data(error in=w537, type=T9 {"Row"=-1, "Column"=-1}, Variant=w539) -> (data=w535:T9, error out=w531:errorcluster)
          n187 = Equal?(x=w535, y=cluster{i32, i32} {-1, -1}) -> (x = y?=w533:bool)
          n188 = call "Substitute Error.vi"("LabVIEW Object"=w540, "error in (no error)"=w531, "Error Code"=5659) -> ("error out"=w532:errorcluster)  [unwired: 8 in]
          n189 = case shown="False" w533 {
            tunnel: w540 -> [w543 w578]
            tunnel: [w542 w577] -> w536
            tunnel: w535 -> [w541 w576]
            frame False {
              n190 = in-place {
                in-place-border: w541 -> [w546]
                n191 = in-place-cluster #11(w543) -> ("Array of Seqs"=w550:refnum<class "Sequence of SBlocks.lvclass">[], "Sequence Index"=w548:i32, "SBlock Index"=w549:i32)
                n192 = Bundle("SBlock Index"=w549, "Sequence Index"=w548) -> (w547:T12)  [unwired: 1 in]
                n193 = Unbundle By Name(w546) -> ("Row"=w552:i32, "Column"=w553:i32)
                n194 = Equal?(x=w546, y=w547) -> (x = y?=w545:bool)
                n195 = case shown="False" w545 {
                  tunnel: w553 -> [w554 _]
                  tunnel: w548 -> [_ _]
                  tunnel: [w555 -1 ("Sequence Index")] -> w544
                  tunnel: w552 -> [w558 _]
                  tunnel: w550 -> [w557 _]
                  tunnel: [w556 -1 ("SBlock Index")] -> w551
                  frame False {
                    n196 = Array Size(array=w557) -> (size(s)=w560:i32)
                    n197 = Less Or Equal?(x=w560, y=w554) -> (x <= y?=w559:bool)
                    n198 = case shown="False" w559 {
                      tunnel: w557 -> [w570 _]
                      tunnel: w554 -> [w562 _]
                      tunnel: [w565 w571] -> w555
                      tunnel: w558 -> [w563 _]
                      tunnel: [w567 w571] -> w556
                      frame False {
                        # "Check if row is in range"
                        n199 = Index Array(array=w570, index=w562) -> (element=w569:refnum<class "Sequence of SBlocks.lvclass">)
                        n200 = call-dynamic "Get Size.vi"("Sequence of SBlocks in"=w569) -> ("size"=w568:i32)  [unwired: 8 in, 2 out]
                        n201 = Less Or Equal?(x=w568, y=w563) -> (x <= y?=w566:bool)
                        n202 = Select(t=-1 ("f"), s=w566, f=w562) -> (s? t:f=w565:i32)
                        n203 = Select(t=-1 ("f"), s=w566, f=w563) -> (s? t:f=w567:i32)
                      }
                      frame True {
                        w571 = -1 ("Row")
                        # "Index out of bounds"
                      }
                    }
                  }
                  frame True {
                  }
                }
                n204 = in-place-cluster #11("Array of Seqs"=w550, "Sequence Index"=w544, "SBlock Index"=w551) -> (w542:refnum<class "Scheduler.lvclass">)
              }
            }
            frame True {
              n205 = Unbundle(w576) -> ("Row"=w575:i32, "Column"=w574:i32)
              n206 = Bundle By Name(cluster=w578, "SBlock Index"=w575, "Sequence Index"=w574) -> (w577:refnum<class "Scheduler.lvclass">)
            }
          }
        }
        frame "Split/Combine Schedules" {
          # "#5660"
          n207 = property class="Scheduler.lvclass"(reference=w586) -> (reference out=w581:refnum<class "Scheduler.lvclass">, "Accessors:Array of Squences"=w580:refnum<class "Sequence of SBlocks.lvclass">[])  [unwired: 1 in, 1 out]
          n208 = Empty Array?(array=w580) -> (empty?=w579:bool)
          n209 = case shown="False" w579 {
            tunnel: w588 -> [w598 _]
            tunnel: w587 -> [w596 w608]
            tunnel: [w591 w607] -> w583
            tunnel: [w590 w608] -> w582
            tunnel: w581 -> [w589 w607]
            frame False {
              n210 = Variant To Data(error in=w596, type=FALSE, Variant=w598) -> (data=w595:bool, error out=w594:errorcluster)
              n211 = case shown="True" w595 {
                tunnel: w589 -> [w602 w606]
                tunnel: [w600 w604] -> w593
                tunnel: w594 -> [w601 w605]
                tunnel: [w599 w603] -> w592
                frame False {
                  # "Parallel mode off, combine all sequences into one"
                  n212 = call-dynamic "Concatenate Sequences.vi"("error in (no error)"=w601, "Scheduler in"=w602) -> ("error out"=w599:errorcluster, "Scheduler out"=w600:refnum<class "Scheduler.lvclass">)  [unwired: 8 in]
                }
                frame True {
                  # "Parallel mode on, split sequences into different columns"
                  n213 = call-dynamic "Split Sequences.vi"("error in (no error)"=w605, "Scheduler in"=w606) -> ("error out"=w603:errorcluster, "Scheduler out"=w604:refnum<class "Scheduler.lvclass">)  [unwired: 8 in]
                }
              }
              n214 = call-dynamic "Estimate Time.vi"("error in (no error)"=w592, "Scheduler in"=w593) -> ("error out"=w590:errorcluster, "Scheduler out"=w591:refnum<class "Scheduler.lvclass">)  [unwired: 8 in]
            }
            frame True {
              # "empty array, we are not doing anything"
            }
          }
          n215 = call "Substitute Error.vi"("LabVIEW Object"=w583, "error in (no error)"=w582, "Error Code"=5660) -> ("error out"=w585:errorcluster)  [unwired: 8 in]
        }
        frame "Reschedule" {
          n216 = Variant To Data(error in=w613, type=refnum<class "Sequence of SBlocks.lvclass"> refnum ("RSequence of SBlocks"), Variant=w618) -> (data=w615:refnum<class "Sequence of SBlocks.lvclass">, error out=w612:errorcluster)
          n217 = Build Array(w615) -> (w614:refnum<class "Sequence of SBlocks.lvclass">[])
          n218 = Bundle By Name(cluster=w616, "Array of Seqs"=w614) -> (w611:refnum<class "Scheduler.lvclass">)
          n219 = call-dynamic "Estimate Time.vi"("error in (no error)"=w612, "Scheduler in"=w611) -> ("error out"=w609:errorcluster, "Scheduler out"=w610:refnum<class "Scheduler.lvclass">)  [unwired: 8 in]
        }
        frame "Load Parameters" {
          n220 = call-dynamic "Load Parameters.vi"("error in (no error)"=w622, "Scheduler in"=w621) -> ("error out"=w619:errorcluster, "Scheduler out"=w620:refnum<class "Scheduler.lvclass">)  [unwired: 8 in]
        }
      }
    }
    frame Error {
    }
  }
  n221 = call-parent "Consumer.vi"("error in (no error)"=w6, "Data"="Data", "Case ID"="Case ID", "uService Template in"=w3) -> ("error out"=→"error out":errorcluster, "uService Template out"=→"Scheduler out":refnum<class "Scheduler.lvclass">)  [unwired: 6 in]
